vi "Func-yyllInitequeue.vi"(7 "max queue size (-1, unlimited)":i32=-1, 8 "error in":errorcluster, 9 "create if not found? (T)":bool=TRUE, 11 "name (unnamed)":string) -> (0 "error out":errorcluster, 1 "created new?":bool, 3 "queue out":refnum<queue>, 4 "remaining elements":cluster{"cmd":string, "data":variant}[](array[cluster]))   [LabVIEW 2017]
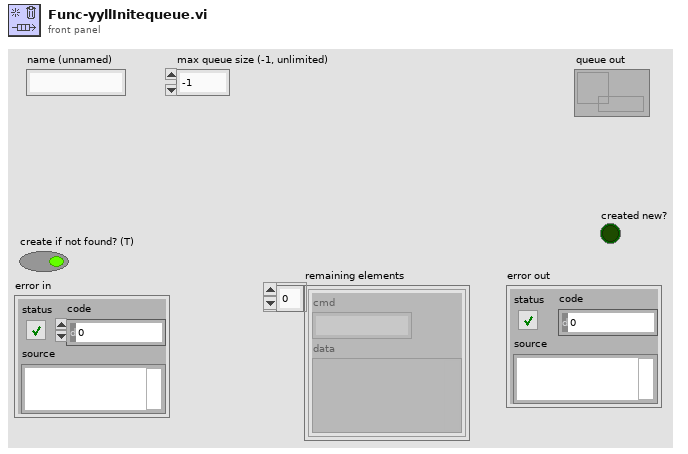
[diagram p1: front panel]
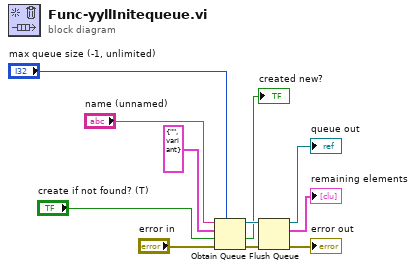
[diagram p0: block diagram]
diagram:
  n1 = Obtain Queue(max queue size (-1, unlimited)="max queue size (-1, unlimited)", name (unnamed)="name (unnamed)", element data type=cluster{"cmd":string, "data":variant} {"cmd"="", "data"=variant}, create if not found? (T)="create if not found? (T)", error in (no error)="error in") -> (queue out=w11:refnum<queue>, created new?=→"created new?":bool, error out=w1:errorcluster)
  n2 = Flush Queue(queue=w11, error in (no error)=w1) -> (queue out=→"queue out":refnum<queue>, remaining elements=→"remaining elements":cluster{"cmd":string, "data":variant}[], error out=→"error out":errorcluster)
